vi "AI_Lookahead.vi"(0 "Ranked":cluster{"Score":dbl, "Row":i32, "Col":i32}[](array[cluster]), 1 "Top K":i32=6, 5 "Grid":enum8{"Empty", "Black", "White"}[][](array[ring])=[[enum."Empty", enum."Empty", enum."Empty", enum."Empty", enum."Empty", enum."Empty", enum."Empty", enum."Empty", enum."Empty", enum."Empty", enum."Empty", enum."Empty", enum."Empty", enum."Empty", enum."Empty"], [enum."Empty", enum."Empty", enum."Empty", enum."Empty", enum."Empty", enum."Empty", enum."Empty", enum."Empty", enum."Empty", enum."Empty", enum."Empty", enum."Empty", enum."Empty", enum."Empty", enum."Empty"], [enum."Empty", enum."Empty", enum."Empty", enum."Empty", enum."Empty", enum."Empty", enum."Empty", enum."Empty", enum."Empty", enum."Empty", enum."Empty", enum."Empty", enum."Empty", enum."Empty", enum."Empty"], [enum."Empty", enum."Empty", enum."Empty", enum."Empty", enum."Empty", enum."Empty", enum."Empty", enum."Empty", enum."Empty", enum."Empty", enum."Empty", enum."Empty", enum."Empty", enum."Empty", enum."Empty"], [enum."Empty", enum."Empty", enum."Empty", enum."Empty", enum."Empty", enum."Empty", enum."Empty", enum."Empty", enum."Empty", enum."Empty", enum."Empty", enum."Empty", enum."Empty", enum."Empty", enum."Empty"], [enum."Empty", enum."Empty", enum."Empty", enum."Empty", enum."Empty", enum."Empty", enum."Empty", enum."Empty", enum."Empty", enum."Empty", enum."Empty", enum."Empty", enum."Empty", enum."Empty", enum."Empty"], [enum."Empty", enum."Empty", enum."Empty", enum."Empty", enum."Empty", enum."Empty", enum."Empty", enum."Empty", enum."Empty", enum."Empty", enum."Empty", enum."Empty", enum."Empty", enum."Empty", enum."Empty"], [enum."Empty", enum."Empty", enum."Empty", enum."Empty", enum."Empty", enum."Empty", enum."Empty", enum."Empty", enum."Empty", enum."Empty", enum."Empty", enum."Empty", enum."Empty", enum."Empty", enum."Empty"], [enum."Empty", enum."Empty", enum."Empty", enum."Empty", enum."Empty", enum."Empty", enum."Empty", enum."Empty", enum."Empty", enum."Empty", enum."Empty", enum."Empty", enum."Empty", enum."Empty", enum."Empty"], [enum."Empty", enum."Empty", enum."Empty", enum."Empty", enum."Empty", enum."Empty", enum."Empty", enum."Empty", enum."Empty", enum."Empty", enum."Empty", enum."Empty", enum."Empty", enum."Empty", enum."Empty"], [enum."Empty", enum."Empty", enum."Empty", enum."Empty", enum."Empty", enum."Empty", enum."Empty", enum."Empty", enum."Empty", enum."Empty", enum."Empty", enum."Empty", enum."Empty", enum."Empty", enum."Empty"], [enum."Empty", enum."Empty", enum."Empty", enum."Empty", enum."Empty", enum."Empty", enum."Empty", enum."Empty", enum."Empty", enum."Empty", enum."Empty", enum."Empty", enum."Empty", enum."Empty", enum."Empty"], [enum."Empty", enum."Empty", enum."Empty", enum."Empty", enum."Empty", enum."Empty", enum."Empty", enum."Empty", enum."Empty", enum."Empty", enum."Empty", enum."Empty", enum."Empty", enum."Empty", enum."Empty"], [enum."Empty", enum."Empty", enum."Empty", enum."Empty", enum."Empty", enum."Empty", enum."Empty", enum."Empty", enum."Empty", enum."Empty", enum."Empty", enum."Empty", enum."Empty", enum."Empty", enum."Empty"], [enum."Empty", enum."Empty", enum."Empty", enum."Empty", enum."Empty", enum."Empty", enum."Empty", enum."Empty", enum."Empty", enum."Empty", enum."Empty", enum."Empty", enum."Empty", enum."Empty", enum."Empty"]], 7 "AI Stone":enum8{"Empty", "Black", "White"}(ring)=enum."White", 9 "Renju":bool=TRUE, 11 "error in":errorcluster) -> (4 "Best":cluster{"Score":dbl, "Row":i32, "Col":i32}, 6 "Value":dbl, 15 "error out":errorcluster)   [LabVIEW 2026]
doc: "Hard/Master 2수 탐색: Ranked 상위 K수(Hard 6, Master 12)를 각각 가상 착수 후 상대의 최선 응수 점수*0.8을 뺀 값이 최대인 수.\n내 수가 5목(>=100000)이면 즉시 그 수."
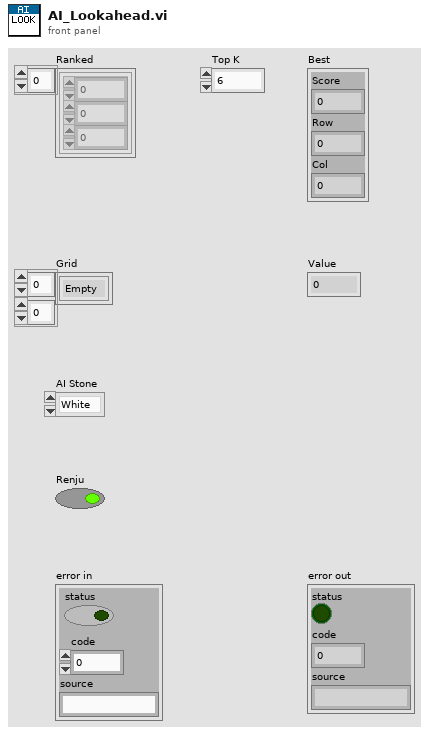
[diagram p1: front panel]
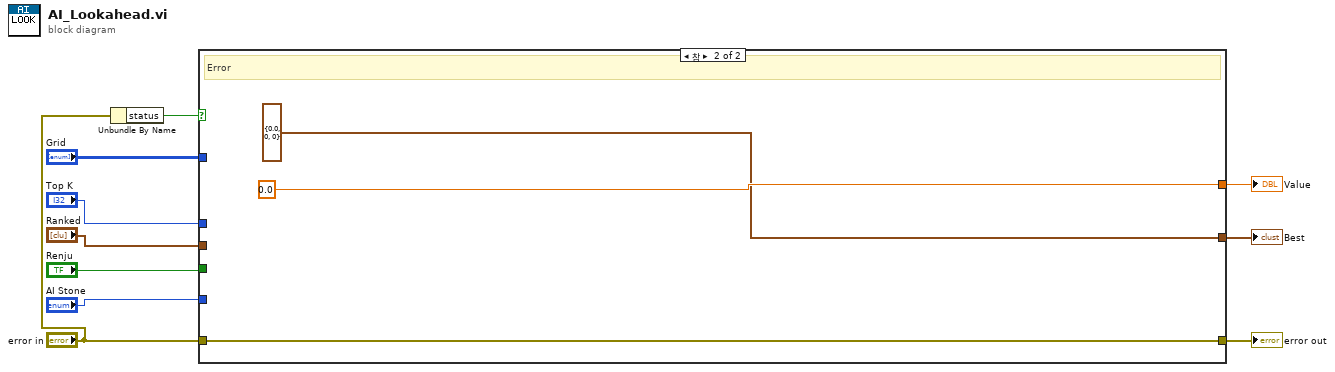
[diagram p0: block diagram]
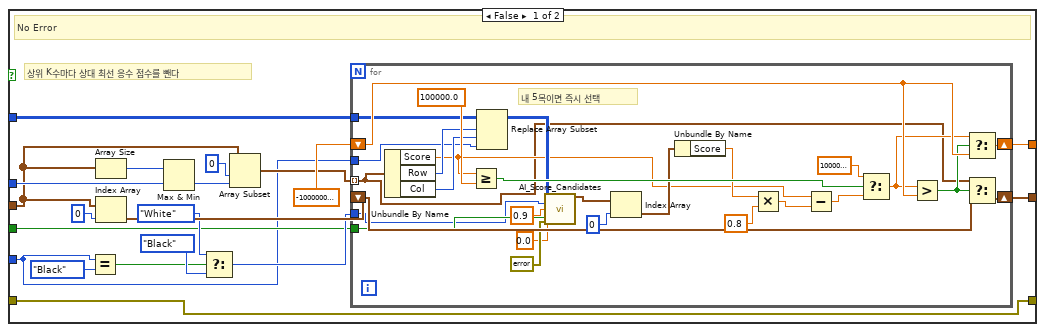
[diagram p2: hidden frame]
diagram:
  n1 = Unbundle By Name("error in") -> ("status"=w7:bool)
  n2 = case shown="참" w7 {
    tunnel: "Ranked" -> [w11 _]
    tunnel: "Grid" -> [w12 _]
    tunnel: "AI Stone" -> [w13 _]
    tunnel: "Renju" -> [w14 _]
    tunnel: "Top K" -> [w15 _]
    tunnel: "error in" -> [w16 w59]
    tunnel: [w29 0.0] -> w9
    tunnel: [w16 w59] -> w10
    tunnel: [w30 cluster{"Score":dbl, "Row":i32, "Col":i32} {"Score"=0.0, "Row"=0, "Col"=0}] -> w8
    frame False {
      # "상위 K수마다 상대 최선 응수 점수를 뺀다"
      # "No Error"
      n3 = Equal?(x=w13, y=enum8{"Empty", "Black", "White"}."Black") -> (x = y?=w18:bool)
      n4 = Array Size(array=w11) -> (size(s)=w22:i32)
      n5 = Index Array(array=w11, index=0) -> (element=w28:cluster{"Score":dbl, "Row":i32, "Col":i32})
      n6 = Max & Min(x=w22, y=w15) -> (min(x,y)=w23:i32)  [unwired: 1 out]
      n7 = Select(t=enum8{"Empty", "Black", "White"}."White", s=w18, f=enum8{"Empty", "Black", "White"}."Black") -> (s? t:f=w21:enum8{"Empty", "Black", "White"})
      n8 = Array Subset(array=w11, index=0, length=w23) -> (w25:cluster{"Score":dbl, "Row":i32, "Col":i32}[])
      n9 = for {
        shift-right: [w56] -> w29
        shift-left: -1000000000000.0 -> [w55]
        tunnel: w12 -> [w31]
        tunnel: w13 -> [w32]
        tunnel: w14 -> [w34]
        shift-right: [w57] -> w30
        shift-left: w28 -> [w58]
        tunnel: w21 -> [w33]
        tunnel: w25 -> [w35] mode=indexing
        # "내 5목이면 즉시 선택"
        n10 = Unbundle By Name(w35) -> ("Score"=w36:dbl, "Row"=w37:i32, "Col"=w38:i32)
        n11 = Greater Or Equal?(x=w36, y=100000.0) -> (x >= y?=w51:bool)
        n12 = Replace Array Subset(array=w31, new element=w32, index (row)=w37, index (col)=w38) -> (w39:enum8{"Empty", "Black", "White"}[][])
        n13 = call "AI_Score_Candidates.vi"("Grid"=w39, "AI Stone"=w33, "Defense Weight"=0.9, "Noise"=0.0, "error in"=errorcluster {"status"=FALSE, "code"=0, "source"=""}, "Renju"=w34) -> ("Ranked"=w43:cluster{"Score":dbl, "Row":i32, "Col":i32}[])  [unwired: 7 in, 2 out]
        n14 = Index Array(array=w43, index=0) -> (element=w45:cluster{"Score":dbl, "Row":i32, "Col":i32})
        n15 = Unbundle By Name(w45) -> ("Score"=w46:dbl)
        n16 = Multiply(x=w46, y=0.8) -> (x*y=w48:dbl)
        n17 = Subtract(x=w36, y=w48) -> (x-y=w49:dbl)
        n18 = Select(t=10000000.0, s=w51, f=w49) -> (s? t:f=w53:dbl)
        n19 = Greater?(x=w53, y=w55) -> (0:w54:bool)
        n20 = Select(t=w53, s=w54, f=w55) -> (s? t:f=w56:dbl)
        n21 = Select(t=w35, s=w54, f=w58) -> (s? t:f=w57:cluster{"Score":dbl, "Row":i32, "Col":i32})
      }
    }
    frame True {
      # "Error"
    }
  }
  "Best" <- w8
  "Value" <- w9
  "error out" <- w10
